vi "ReferenceMove.vi"(6 "New command":bool, 8 "error in (no error)":errorcluster, 10 "Array":dbl[](array[numeric]), 11 "SoftmotionAxis in":refnum<class "SoftmotionAxis.lvclass">) -> (0 "error out":errorcluster, 3 "SoftmotionAxis out":refnum<class "SoftmotionAxis.lvclass">)   [LabVIEW 2017, in "SoftmotionAxis.lvclass"]
uses:
  SoftmotionAxis.lvclass
  <vilib>/Motion/Express/_s/nimc.ex.stopMove.stop.axis.modeDecelerate.vi
  <vilib>/Motion/BlockNode/FB.NIMotion.xnode
  <resource>/objmgr/nimotion.rc
  Utilities/WordManipulationLibrary.lvlib
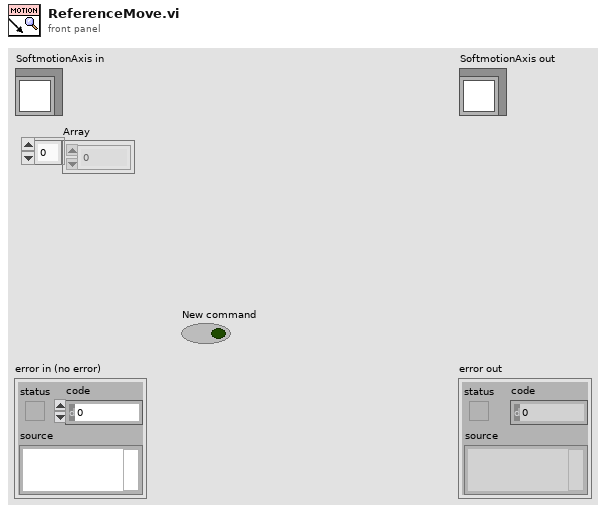
[diagram p1: front panel]
types:
  T1 = typedef "WordManipulationLibrary.lvlib/Parameters_Reference.ctl" = cluster{"Reference Move Mode":i32, "Start Search Forward":bool, "Stop on FWD Edge":bool, "Approach Forward":bool, "Velocity":dbl, "Acceleration":dbl}
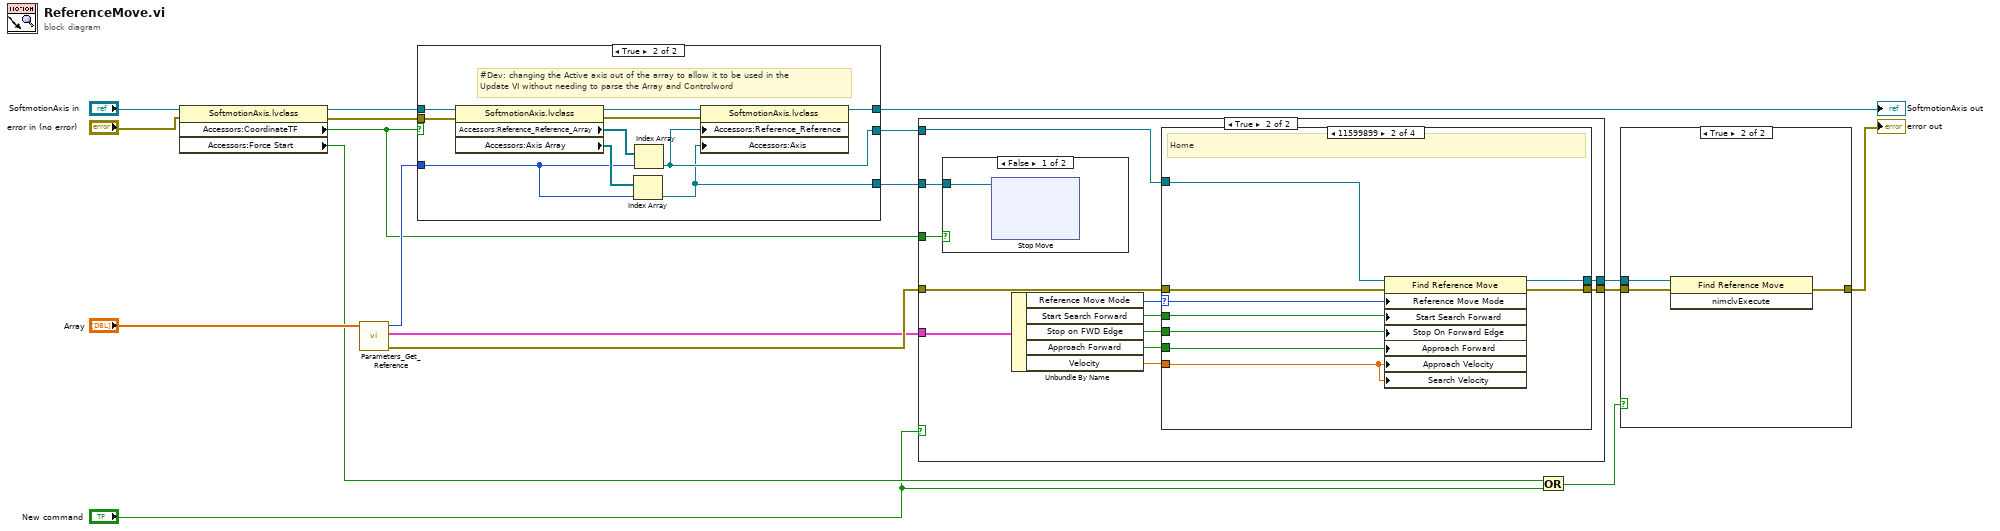
[diagram p0: block diagram]
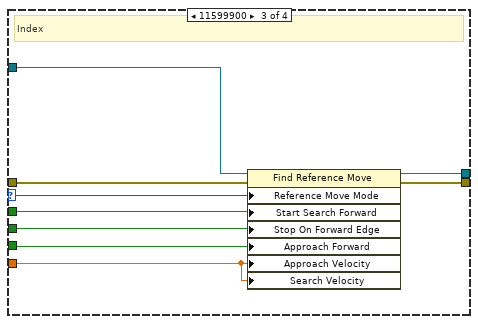
[diagram p5: hidden frame]
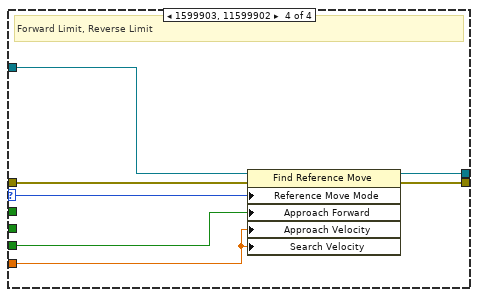
[diagram p6: hidden frame]
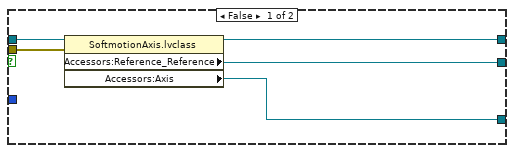
[diagram p7: hidden frame]
diagram:
  n1 = property class="SoftmotionAxis.lvclass"(reference="SoftmotionAxis in", error in="error in (no error)") -> (reference out=w11:refnum<class "SoftmotionAxis.lvclass">, error out=w10:errorcluster, "Accessors:CoordinateTF"=w1:bool, "Accessors:Force Start"=w8:bool)
  n2 = call "Parameters_Get_Reference.vi"("Parameters"="Array") -> ("error out"=w6:errorcluster, "Reference Move Parameters"=w5:T1, "Axis to command"=w4:i32)  [unwired: 8 in]
  n3 = case shown="True" w1 {
    tunnel: [w23 w29] -> w15
    tunnel: [w22 w27] -> w7
    tunnel: w11 -> [w21 w33]
    tunnel: w10 -> [w20 w32]
    tunnel: w4 -> [_ w25]
    tunnel: [w19 w24] -> w2
    frame False {
      n4 = property class="SoftmotionAxis.lvclass"(reference=w21, error in=w20) -> (reference out=w23:refnum<class "SoftmotionAxis.lvclass">, "Accessors:Reference_Reference"=w22:refnum<k20>, "Accessors:Axis"=w19:refnum<k21>)  [unwired: 1 out]
    }
    frame True {
      # "#Dev: changing the Active axis out of the array to allow it to be used in the \nUpdate VI without needing to parse the Array and Controlword"
      n5 = property class="SoftmotionAxis.lvclass"(reference=w33, error in=w32) -> (reference out=w30:refnum<class "SoftmotionAxis.lvclass">, error out=w28:errorcluster, "Accessors:Reference_Reference_Array"=w31:refnum<k20>[], "Accessors:Axis Array"=w26:refnum<k21>[])
      n6 = Index Array(array=w26, index=w25) -> (element=w24:refnum<k21>)
      n7 = Index Array(array=w31, index=w25) -> (element=w27:refnum<k20>)
      n8 = property class="SoftmotionAxis.lvclass"(reference=w30, error in=w28, "Accessors:Reference_Reference"=w27, "Accessors:Axis"=w24) -> (reference out=w29:refnum<class "SoftmotionAxis.lvclass">)  [unwired: 1 out]
    }
  }
  "SoftmotionAxis out" <- w15
  n9 = case shown="True" "New command" {
    tunnel: [w35 w47] -> w13
    tunnel: [w34 w46] -> w12
    tunnel: w7 -> [w35 w45]
    tunnel: w6 -> [w34 w40]
    tunnel: w5 -> [_ w38]
    tunnel: w1 -> [_ w37]
    tunnel: w2 -> [_ w36]
    frame False {
    }
    frame True {
      n10 = case shown="False" w37 {
        tunnel: w36 -> [w48 _]
        frame False {
          n11 = xnode ("Stop Move")("resource"=w48) -> ()  [unwired: 2 in, 3 out]
        }
        frame True {
        }
      }
      n12 = Unbundle By Name(w38) -> ("Reference Move Mode"=w44:i32, "Start Search Forward"=w42:bool, "Stop on FWD Edge"=w41:bool, "Approach Forward"=w43:bool, "Velocity"=w39:dbl)
      n13 = case shown="11599899" w44 {
        selector: w44 -> [_ w62 w71 w79]
        tunnel: w45 -> [w57 w67 w76 w83]
        tunnel: w39 -> [_ w59 w68 w77]
        tunnel: [w57 w66 w75 w82] -> w47
        tunnel: [w58 w65 w74 w81] -> w46
        tunnel: w43 -> [_ w61 w70 w80]
        tunnel: w42 -> [_ w64 w73 _]
        tunnel: w41 -> [_ w63 w72 _]
        tunnel: w40 -> [w58 w60 w69 w78]
        frame 0, Default {
        }
        frame 11599899 {
          # "Home"
          n14 = property class="Find Reference Move"(reference=w67, error in=w60, "Reference Move Mode"=w62, "Start Search Forward"=w64, "Stop On Forward Edge"=w63, "Approach Forward"=w61, "Approach Velocity"=w59, "Search Velocity"=w59) -> (reference out=w66:refnum<k20>, error out=w65:errorcluster)
        }
        frame 11599900 {
          # "Index"
          n15 = property class="Find Reference Move"(reference=w76, error in=w69, "Reference Move Mode"=w71, "Start Search Forward"=w73, "Stop On Forward Edge"=w72, "Approach Forward"=w70, "Approach Velocity"=w68, "Search Velocity"=w68) -> (reference out=w75:refnum<k20>, error out=w74:errorcluster)
        }
        frame 1599903, 11599902 {
          # "Forward Limit, Reverse Limit"
          n16 = property class="Find Reference Move"(reference=w83, error in=w78, "Reference Move Mode"=w79, "Approach Forward"=w80, "Approach Velocity"=w77, "Search Velocity"=w77) -> (reference out=w82:refnum<k20>, error out=w81:errorcluster)
        }
      }
    }
  }
  n17 = Or(x=w8, y="New command") -> (x .or. y?=w9:bool)
  n18 = case shown="True" w9 {
    tunnel: [w84 w87] -> w17
    tunnel: w13 -> [_ w86]
    tunnel: w12 -> [w84 w85]
    frame False {
    }
    frame True {
      n19 = invoke class="Find Reference Move" method="nimclvExecute"(reference=w86, error in=w85) -> (error out=w87:errorcluster)  [unwired: 1 in, 2 out]
    }
  }
  "error out" <- w17
